vi "Read CIF Subscriber Refnum.vi"(8 "error in (no error)":errorcluster, 11 "CIF_Iceoryx_PCAP_Universal in":refnum<class "CIF_Iceoryx_PCAP_Universal.lvclass">) -> (0 "error out":errorcluster, 2 "CIF Subscriber Refnum":T1 {"refnum" format="%.0x"}, 3 "CIF_Iceoryx_PCAP_Universal out":refnum<class "CIF_Iceoryx_PCAP_Universal.lvclass">)   [LabVIEW 2021, in "CIF_Iceoryx_PCAP_Universal.lvclass"]
uses:
  CIF_Iceoryx_PCAP_Universal.lvclass
  <vilib>/CIF Foundation/CIF Iceoryx/Refnum/Typedef/CIF Subscriber Refnum.ctl
  CIF_Iceoryx_PCAP_Universal.lvclass/CIF_Iceoryx_PCAP_Universal.ctl
  <vilib>/CIF Foundation/CIF Iceoryx/Iceoryx.lvlib
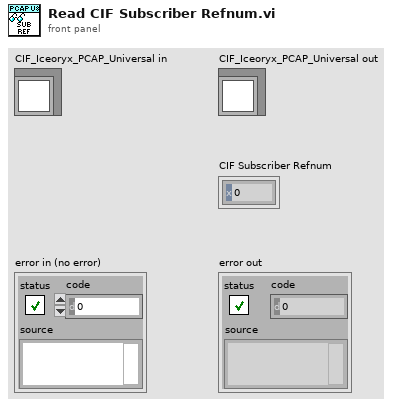
[diagram p1: front panel]
types:
  T1 = typedef "Iceoryx.lvlib/CIF Subscriber Refnum.ctl" = cluster{"refnum":u64, "CIF Sub":enum8{"cifsub"}}
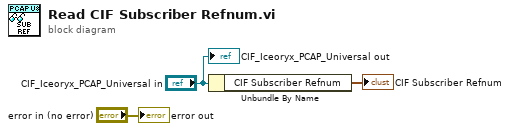
[diagram p0: block diagram]
diagram:
  n1 = Unbundle By Name("CIF_Iceoryx_PCAP_Universal in") -> ("CIF Subscriber Refnum"=→"CIF Subscriber Refnum":T1)
  "error out" <- "error in (no error)"
  "CIF_Iceoryx_PCAP_Universal out" <- "CIF_Iceoryx_PCAP_Universal in"
